vi "Time Assigned TableZ.vi"(8 "Time Probability":dbl[][](array[numeric]), 9 "current":dbl[](array[numeric]), 10 "time":dbl[](array[numeric]), 11 "Assigned Time Profile plus":T2) -> (3 "Time Profile Table P":string[][](table) caption="Time Table")   [LabVIEW 2018]
panel:
  in  "Table Tag 2":T1
  out "サイズ 3":i32
  out "サイズ 7":i32
  out "配列":string[][](array[string])
  out "要素":i32
  out "サイズ 2":i32
  out "サイズ":i32[](array[numeric])
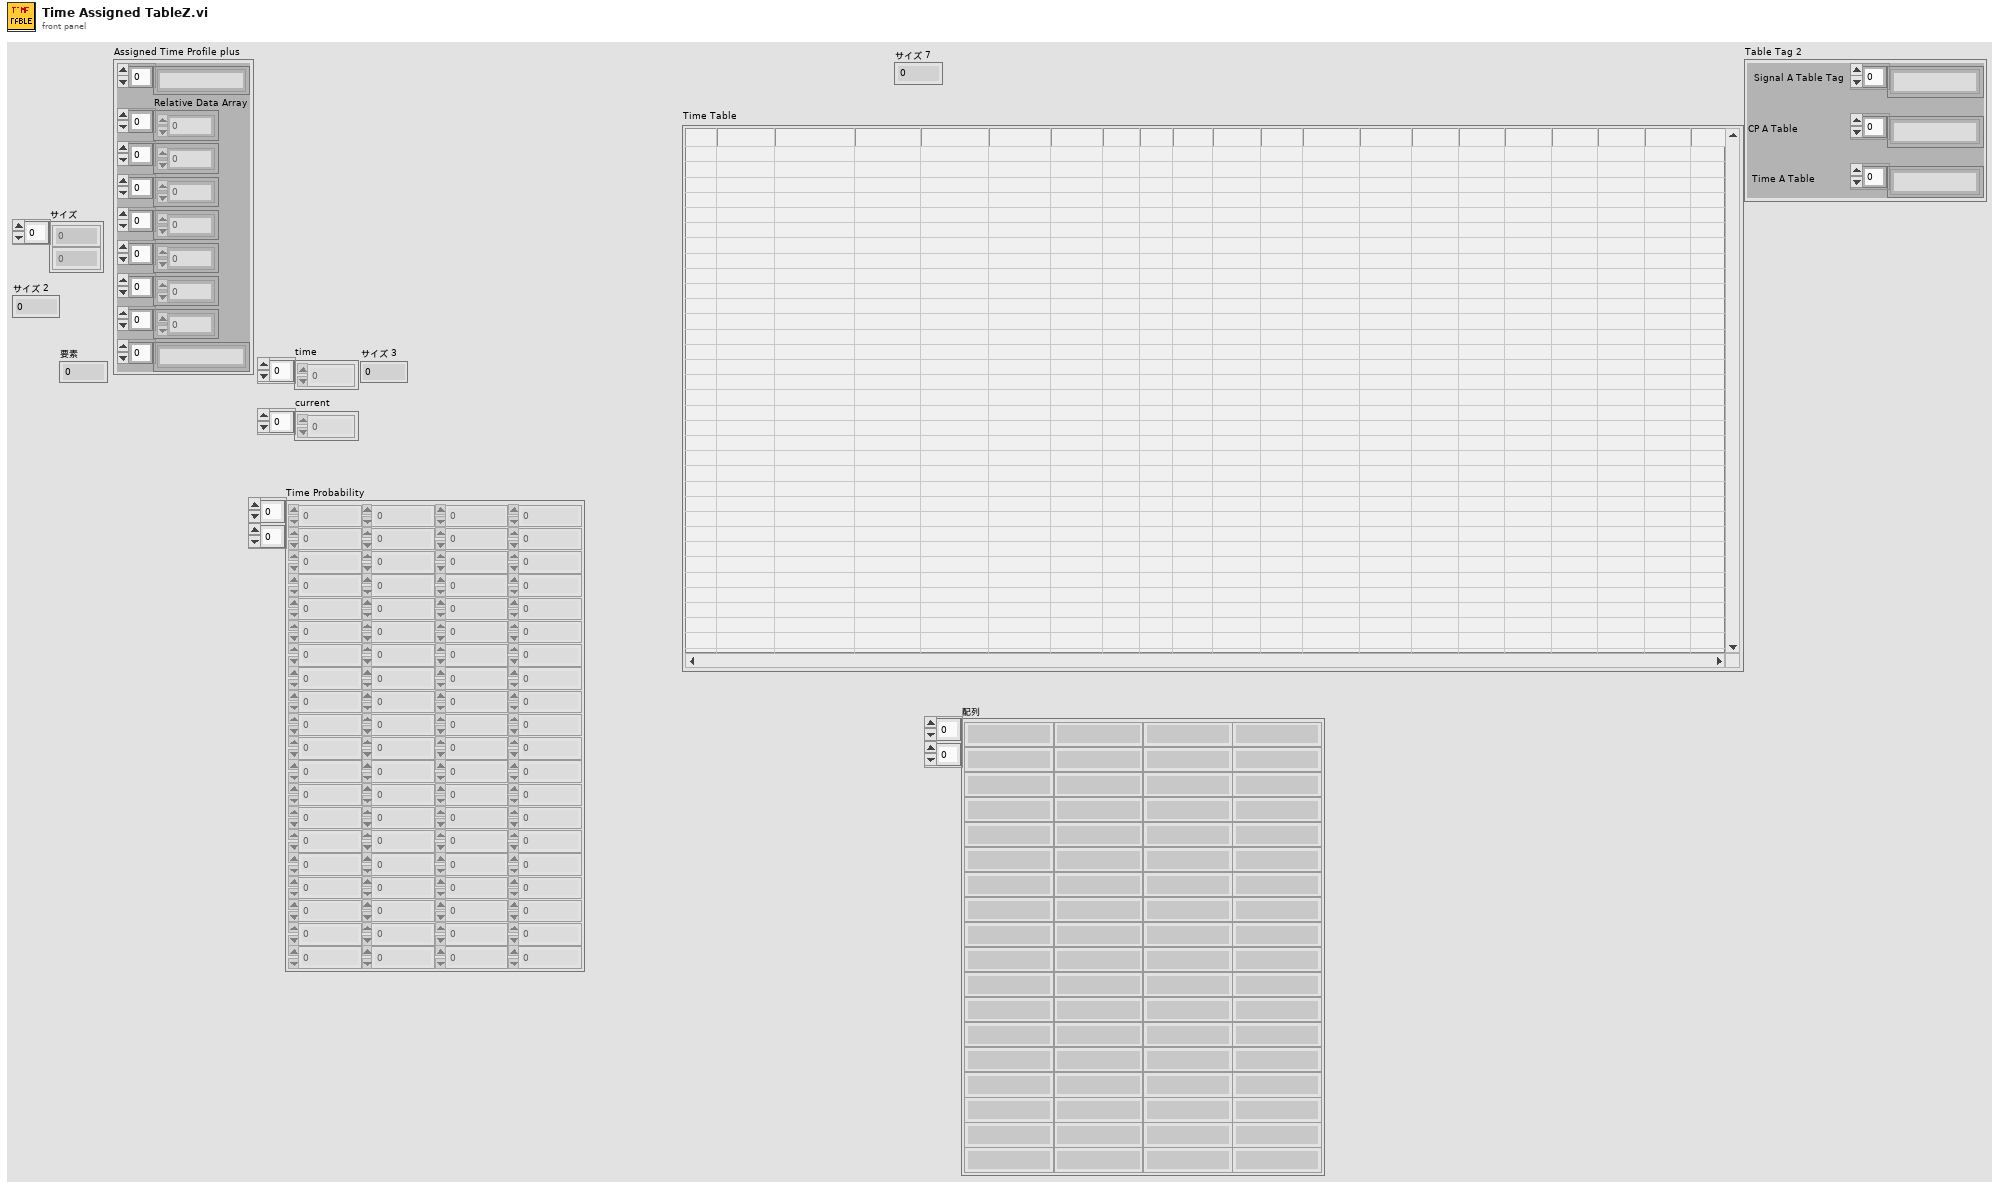
[diagram p1: front panel]
types:
  T1 = cluster{"Signal A Table Tag":string[], "CP A Table":string[], "Time A Table":string[]}
  T2 = cluster{string[], "Relative Data Array":dbl[], dbl[], dbl[], dbl[], i32[], i32[], i32[], string[]}
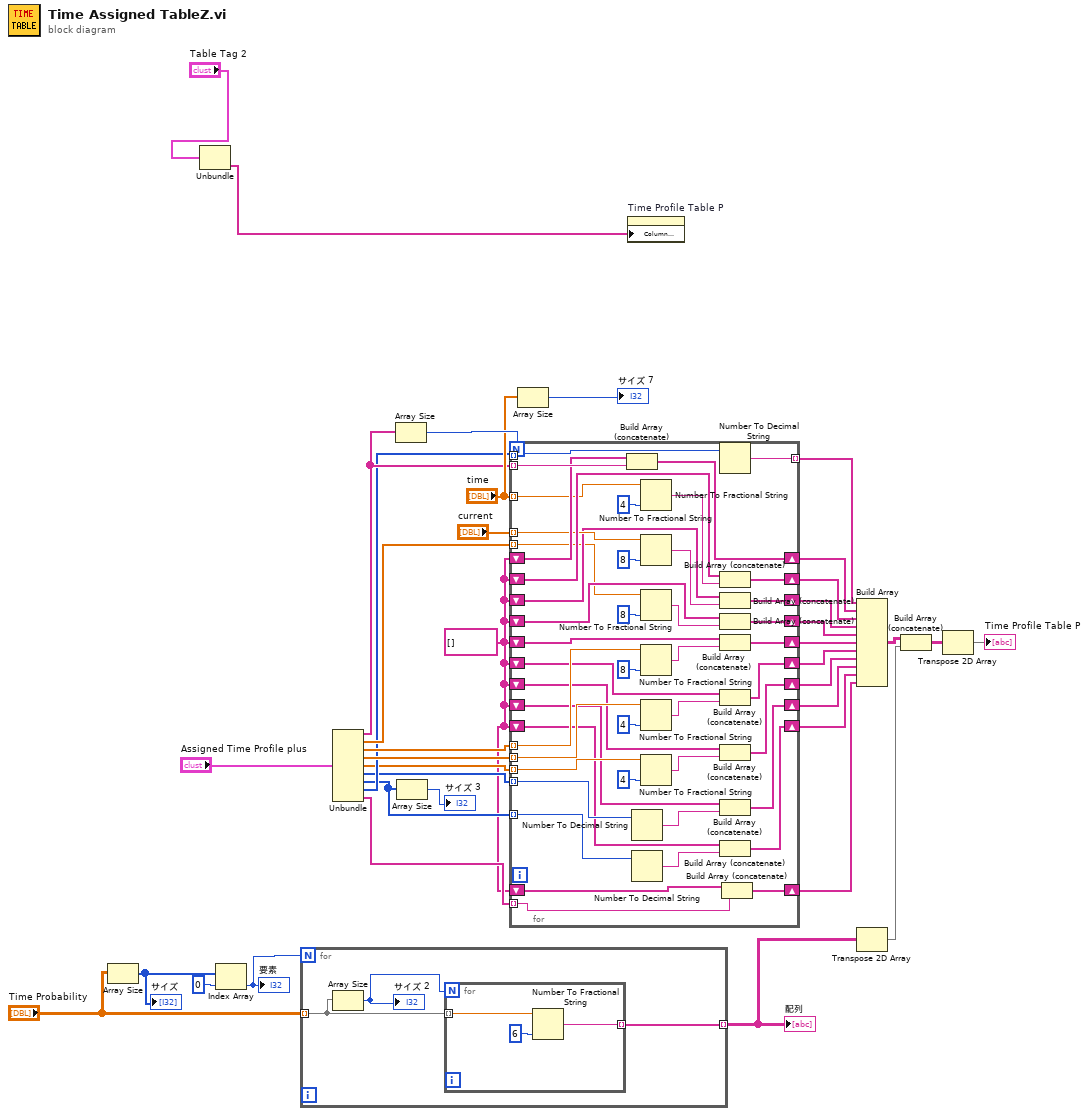
[diagram p0: block diagram]
diagram:
  w4 = string[] []
  n1 = Array Size(array="Time Probability") -> (size(s)=w38:i32[])
  "サイズ" <- w38
  n2 = Unbundle("Table Tag 2") -> ("Time A Table"=w2:string[])  [unwired: 2 out]
  n3 = Index Array(array=w38, index=0 ("指標")) -> (element=w36:i32)
  "要素" <- w36
  n4 = for {
    N: w36 -> [_]
    tunnel: "Time Probability" -> [w40] mode=indexing
    tunnel: [w39] -> w25 mode=indexing
    n5 = Array Size(array=w40) -> (size(s)=w41:i32)
    "サイズ 2" <- w41
    n6 = for {
      N: w41 -> [_]
      tunnel: w40 -> [w44] mode=indexing
      tunnel: [w43] -> w39 mode=indexing
      n7 = Number To Fractional String(number=w44, precision (6)=i16 6 ("精度（6）")) -> (F-format string=w43:string)  [unwired: 2 in]
    }
  }
  "配列" <- w25
  n8 = Unbundle("Assigned Time Profile plus") -> (w13:string[], "Relative Data Array"=w12:dbl[], w11:dbl[], w10:dbl[], w6:dbl[], w7:i32[], w8:i32[], w9:i32[], w5:string[])
  n9 = Array Size(array=w13) -> (size(s)=w19:i32)
  n10 = Array Size(array=w8) -> (size(s)=→"サイズ 3":i32)
  n11 = for {
    N: w19 -> [_]
    tunnel: w13 -> [w90] mode=indexing
    tunnel: w12 -> [w73] mode=indexing
    tunnel: "time" -> [w83] mode=indexing
    tunnel: "current" -> [w79] mode=indexing
    tunnel: w11 -> [w67] mode=indexing
    tunnel: w10 -> [w62] mode=indexing
    tunnel: w6 -> [w58] mode=indexing
    tunnel: w7 -> [w54] mode=indexing
    tunnel: w8 -> [w53] mode=indexing
    shift-right: [w89] -> w34
    shift-left: w4 -> [w88]
    shift-right: [w85] -> w21
    shift-left: w4 -> [w84]
    shift-right: [w80] -> w33
    shift-left: w4 -> [w78]
    shift-right: [w75] -> w32
    shift-left: w4 -> [w74]
    shift-right: [w69] -> w31
    shift-left: w4 -> [w68]
    shift-right: [w63] -> w30
    shift-left: w4 -> [w61]
    shift-right: [w60] -> w29
    shift-left: w4 -> [w59]
    shift-right: [w56] -> w28
    shift-left: w4 -> [w55]
    shift-right: [w51] -> w27
    shift-left: w4 -> [w50]
    tunnel: w9 -> [w49] mode=indexing
    tunnel: [w48] -> w15 mode=indexing
    tunnel: w5 -> [w47] mode=indexing
    shift-right: [w46] -> w3
    shift-left: w4 -> [w45]
    n12 = Build Array (concatenate)(w88, w90) -> (w89:string[])
    n13 = Number To Decimal String(number=w54) -> (decimal integer string=w57:string)  [unwired: 1 in]
    n14 = Number To Decimal String(number=w53) -> (decimal integer string=w52:string)  [unwired: 1 in]
    n15 = Number To Fractional String(number=w83, precision (6)=i16 4 ("精度（6）")) -> (F-format string=w86:string)  [unwired: 2 in]
    n16 = Number To Fractional String(number=w79, precision (6)=i16 8 ("精度（6）")) -> (F-format string=w81:string)  [unwired: 2 in]
    n17 = Number To Fractional String(number=w73, precision (6)=i16 8 ("精度（6）")) -> (F-format string=w76:string)  [unwired: 2 in]
    n18 = Number To Fractional String(number=w67, precision (6)=i16 8 ("精度（6）")) -> (F-format string=w70:string)  [unwired: 2 in]
    n19 = Number To Fractional String(number=w62, precision (6)=i16 4 ("精度（6）")) -> (F-format string=w65:string)  [unwired: 2 in]
    n20 = Number To Fractional String(number=w58, precision (6)=i16 4 ("精度（6）")) -> (F-format string=w64:string)  [unwired: 2 in]
    n21 = Number To Decimal String(number=w49) -> (decimal integer string=w48:string)  [unwired: 1 in]
    n22 = Build Array (concatenate)(w84, w86) -> (w85:string[])
    n23 = Build Array (concatenate)(w78, w81) -> (w80:string[])
    n24 = Build Array (concatenate)(w74, w76) -> (w75:string[])
    n25 = Build Array (concatenate)(w68, w70) -> (w69:string[])
    n26 = Build Array (concatenate)(w61, w65) -> (w63:string[])
    n27 = Build Array (concatenate)(w59, w64) -> (w60:string[])
    n28 = Build Array (concatenate)(w55, w57) -> (w56:string[])
    n29 = Build Array (concatenate)(w50, w52) -> (w51:string[])
    n30 = Build Array (concatenate)(w45, w47) -> (w46:string[])
  }
  n31 = Array Size(array="time") -> (size(s)=→"サイズ 7":i32)
  n32 = property on="Time Profile Table P" class="Tbl (strict)"("Column Headers[]"=w2) -> ()  [unwired: 2 in, 2 out]
  n33 = Build Array(w15, w34, w21, w33, w32, w31, w30, w29, w28, w27, w3) -> (w22:string[][])
  n34 = Transpose 2D Array(2D array=w25) -> (transposed array=w23:string[][])
  n35 = Build Array (concatenate)(w22, w23) -> (w26:string[][])
  n36 = Transpose 2D Array(2D array=w26) -> (transposed array=→"Time Profile Table P":string[][])
